vi "Test Context Survives Creator Stopping.vi"(8 "error in (no error)":errorcluster) -> (0 "error out":errorcluster)   [LabVIEW 2019, in "RemoteControl.ZMQ.Tests.lvclass"]
uses:
  RemoteControl.ZMQ.Tests.lvclass
  Test Helper - Open and Close Client.vi
  <vilib>/addons/_JKI Toolkits/Caraya/classes/Test/Test.lvclass
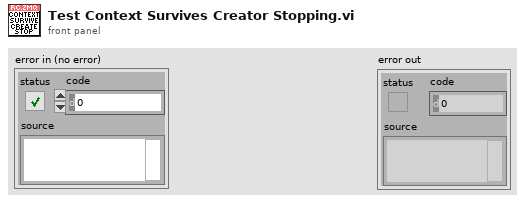
[diagram p1: front panel]
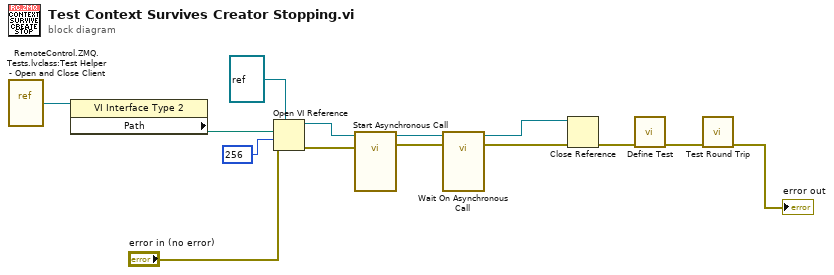
[diagram p0: block diagram]
diagram:
  n1 = vi-ref "RemoteControl.ZMQ.Tests.lvclass:Test Helper - Open and Close Client.vi"() -> (w12:refnum<vi>)
  n2 = property class="VI Interface Type 2"(reference=w12) -> ("Path"=w11:path)  [unwired: 1 in, 2 out]
  n3 = Open VI Reference(type specifier VI Refnum (for type only)=refnum<vi> refnum, vi path=w11, options=256, error in (no error)="error in (no error)") -> (vi reference=w10:refnum<vi>, error out=w9:errorcluster)  [unwired: 2 in]
  n4 = call-by-ref "Start Asynchronous Call"(reference=w10, error in=w9) -> (reference out=w8:refnum<vi>, error out=w7:errorcluster)  [unwired: 11 in, 1 out]
  n5 = call-by-ref "Wait On Asynchronous Call"(reference=w8, error in=w7) -> (reference out=w5:refnum<vi>, error out=w6:errorcluster)  [unwired: 11 in, 1 out]
  n6 = Close Reference(reference=w5, error in (no error)=w6) -> (error out=w4:errorcluster)
  n7 = call <vilib>:"Define Test.vi"("error in (no error)"=w4) -> ("error out"=w3:errorcluster)  [unwired: 9 in, 1 out]
  n8 = call "Test Round Trip.vi"("error in (no error)"=w3) -> ("error out"=→"error out":errorcluster)  [unwired: 10 in]
